vi "BoolCmd_Recv.vi"(7 "Command Name":string) -> (0 "error out":errorcluster, 3 "New Request":bool)   [LabVIEW 2019, in "Trajectory_Library.lvlib"]
uses:
  Trajectory_Library.lvlib
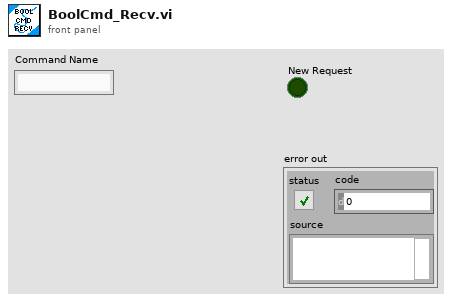
[diagram p1: front panel]
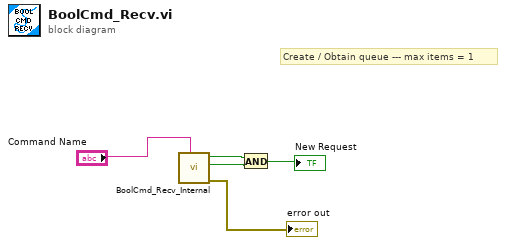
[diagram p0: block diagram]
diagram:
  # "Create / Obtain queue --- max items = 1"
  n1 = call "BoolCmd_Recv_Internal.vi"("Command Name"="Command Name") -> ("error out"=→"error out":errorcluster, "New Request"=w4:bool, "Newest Value"=w5:bool)  [unwired: 8 in]
  n2 = And(x=w5, y=w4) -> (x .and. y?=→"New Request":bool)
